vi "Execute Lua Script.vi"(4 "nresults":i32=-1, 6 "nargs":i32=-1, 9 "lua script":string, 10 "error in (no error)":errorcluster, 11 "Lua in":refnum<class "Lua.lvclass">) -> (2 "error out":errorcluster, 3 "Lua out":refnum<class "Lua.lvclass">)   [LabVIEW 2020, in "Lua for LabVIEW.lvlib" / "Lua.lvclass"]
doc: "Load and execute a Lua script. Specify the number of return values expected from the script using the nresults argument. For example, to return a number from a script, the script could end with:\n\n...\nreturn my_number_result\n\nIf nargs = -1, then any values on the stack at the time of the call will be passed to the script.\nIf nresult = -1, then all values returned from the script will be left on the stack after the call."
uses:
  Lua.lvclass
  Lua.lvclass/Lua.ctl
  lib/lua.dll/lua_type.vi
  lib/lua.dll/lua_tolstring.vi
  lib/lua.dll/lua_pop.vi
  lib/lua.dll/lua_settop.vi
  lib/lua.dll/lua.dll.lvlib
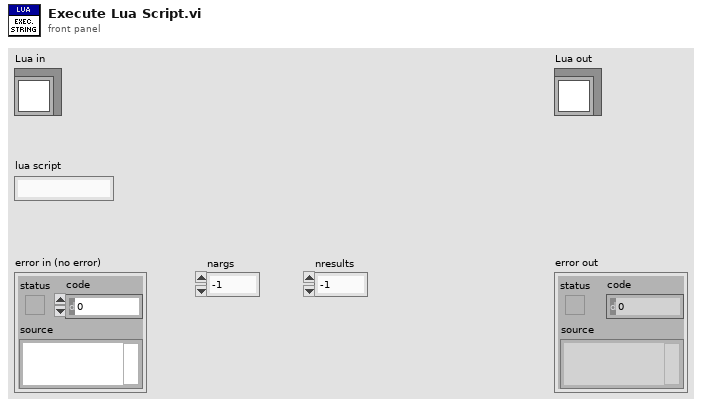
[diagram p1: front panel]
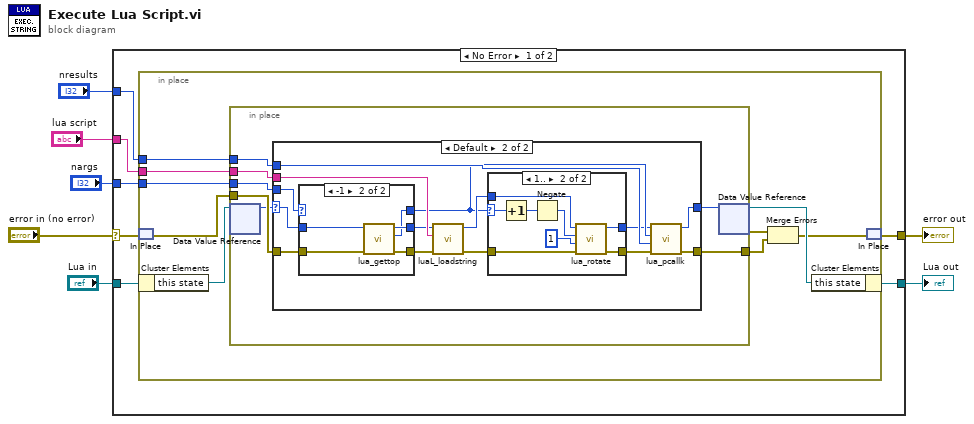
[diagram p0: block diagram]
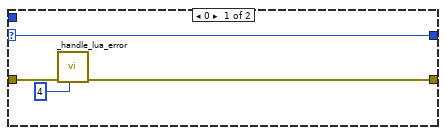
[diagram p2: hidden frame]
diagram:
  n1 = case shown="No Error" "error in (no error)" {
    selector: "error in (no error)" -> [w11 w68]
    tunnel: [w12 w68] -> w4
    tunnel: [w13 w67] -> w7
    tunnel: "Lua in" -> [w14 w67]
    tunnel: "nargs" -> [w10 _]
    tunnel: "nresults" -> [w9 _]
    tunnel: "lua script" -> [w8 _]
    frame No Error {
      n2 = in-place {
        in-place-border: w10 -> [w22]
        in-place-border: w9 -> [w21]
        in-place-border: w8 -> [w20]
        n3 = in-place-match #1(w11) -> (w23:errorcluster)
        n4 = in-place-cluster #2(w14) -> ("this state"=w19:refnum<data-value>)
        n5 = in-place {
          in-place-border: w23 -> [w30]
          in-place-border: w22 -> [w29]
          in-place-border: w21 -> [w28]
          in-place-border: w20 -> [w27]
          in-place-border: [w24] -> w16
          n6 = in-place-dvr #3(w19) -> (w26:u64)  [unwired: 1 out]
          n7 = case shown="Default" w26 {
            selector: w26 -> [w34 w39]
            tunnel: [w34 w48] -> w25
            tunnel: w30 -> [w31 w36]
            tunnel: [w32 w46] -> w24
            tunnel: w29 -> [_ w41]
            tunnel: w28 -> [_ w47]
            tunnel: w27 -> [_ w43]
            frame 0 {
              n8 = call "_handle_lua_error.vi"("lua status"=4 ("lua_load errcode"), "error in (no error)"=w31) -> ("error out"=w32:errorcluster)  [unwired: 9 in]
            }
            frame Default {
              n9 = case shown="-1" w41 {
                selector: w41 -> [w51 _]
                tunnel: [w51 w54] -> w40
                tunnel: w39 -> [w49 w56]
                tunnel: [w49 w55] -> w38
                tunnel: [w50 w53] -> w37
                tunnel: w36 -> [w50 w52]
                frame Default {
                }
                frame -1 {
                  n10 = call "lua_gettop.vi"("error in (no error)"=w52, "lua_state_p"=w56) -> ("error out"=w53:errorcluster, "index"=w54:i32, "lua_state_p out"=w55:u64)  [unwired: 7 in]
                }
              }
              n11 = call "luaL_loadstring.vi"("error in (no error)"=w37, "lua chunk"=w43, "lua_state_p"=w38) -> ("error out"=w45:errorcluster, "lua_state_p out"=w44:u64)  [unwired: 7 in]
              n12 = case shown="1.." w40 {
                selector: w40 -> [_ w60]
                tunnel: w44 -> [w58 w66]
                tunnel: [w58 w65] -> w35
                tunnel: [w57 w64] -> w42
                tunnel: w45 -> [w57 w63]
                frame Default {
                }
                frame 1.. {
                  n13 = Increment(x=w60) -> (x+1=w59:i32)
                  n14 = Negate(x=w59) -> (-x=w62:i32)
                  n15 = call "lua_rotate.vi"("error in (no error)"=w63, "n"=1, "index"=w62, "lua_state_p"=w66) -> ("error out"=w64:errorcluster, "lua_state_p out"=w65:u64)  [unwired: 6 in]
                }
              }
              n16 = call "lua_pcallk.vi"("error in (no error)"=w42, "nresults"=w47, "nargs"=w40, "lua_state_p"=w35) -> ("error out"=w46:errorcluster, "lua_state_p out"=w48:u64)  [unwired: 6 in]
            }
          }
          n17 = in-place-dvr #3(w25) -> (w18:refnum<data-value>, w17:errorcluster)
        }
        n18 = Merge Errors(w17, w16) -> (w15:errorcluster)
        n19 = in-place-cluster #2("this state"=w18) -> (w13:refnum<class "Lua.lvclass">)
        n20 = in-place-match #1(w15) -> (w12:errorcluster)
      }
    }
    frame Error {
    }
  }
  "error out" <- w4
  "Lua out" <- w7
